vi "Index VI.vi"(6 "DBMap":refnum<class "DBMap.lvclass">, 7 "VI to analyze":path=path "C:/Projects/DMC/VISight/Source/Analyzer/Fibonacci.vi", 8 "error in (no error)":errorcluster, 9 "Valid Terminals Set":set{string}(c389)={"ControlTerminal", "OverridableParameterTerminal", "Terminal"}, 10 "AtomicSet":refnum<class "DBSet.lvclass">) -> (0 "error out":errorcluster, 3 "File Data":T1)   [LabVIEW 2020]
uses:
  DBSet/DBSet.lvclass
  DBMap/DBMap.lvclass
  <vilib>/Utility/miscctls.llb/LVMapReplaceAction.ctl
  <vilib>/Utility/traverseref.llb/VI Scripting - Traverse.lvlib
  <vilib>/Utility/traverseref.llb/TRef TravTarget.ctl
  <vilib>/security/Message Digest/API/NI_Message Digest API.lvlib
  File Metadata.ctl
  Source to Sink Array.ctl
  Node.ctl
  <vilib>/security/Message Digest/API/Instances/File/SHA-256 File Checksum.vi
  File Data.ctl
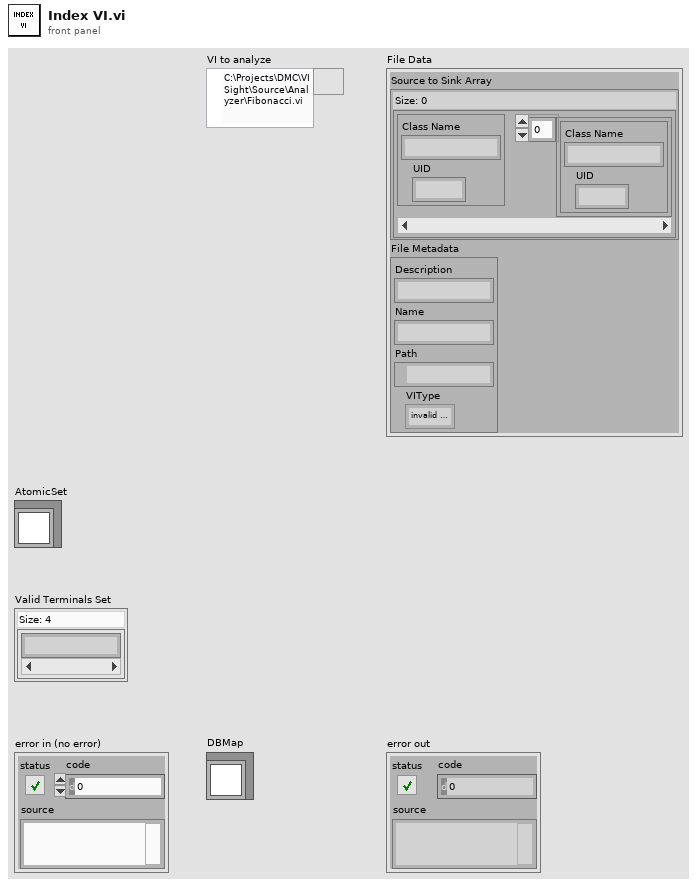
[diagram p1: front panel]
types:
  T1 = typedef "File Data.ctl" = cluster{"Source to Sink Array":T2, "File Metadata":T4}
  T2 = typedef "Source to Sink Array.ctl" = map{T3, T3[]}
  T3 = typedef "Node.ctl" = cluster{"Class Name":string, "UID":i32}
  T4 = typedef "File Metadata.ctl" = cluster{"Description":string, "Name":string, "Path":path, "VIType":enum32{"invalid VI type", "Standard VI", "Control VI", "Global VI", "Polymorphic VI", "Configuration VI", "SubSystem", "Facade VI", "Method VI", "Statechart Diagram VI"}}
  T5 = typedef "TRef TravTarget.ctl" = enum16{"FP", "BD", "Other"}
  T6 = typedef "LVMapReplaceAction.ctl" = enum32{"Modify Entry only if found", "Add or Modify Entry", "Delete Entry"}
  T7 = enum32{"invalid VI type", "Standard VI", "Control VI", "Global VI", "Polymorphic VI", "Configuration VI", "SubSystem", "Facade VI", "Method VI", "Statechart Diagram VI"}
  T8 = cluster{"ClassName":string, "Caption":string, "UID":i32}
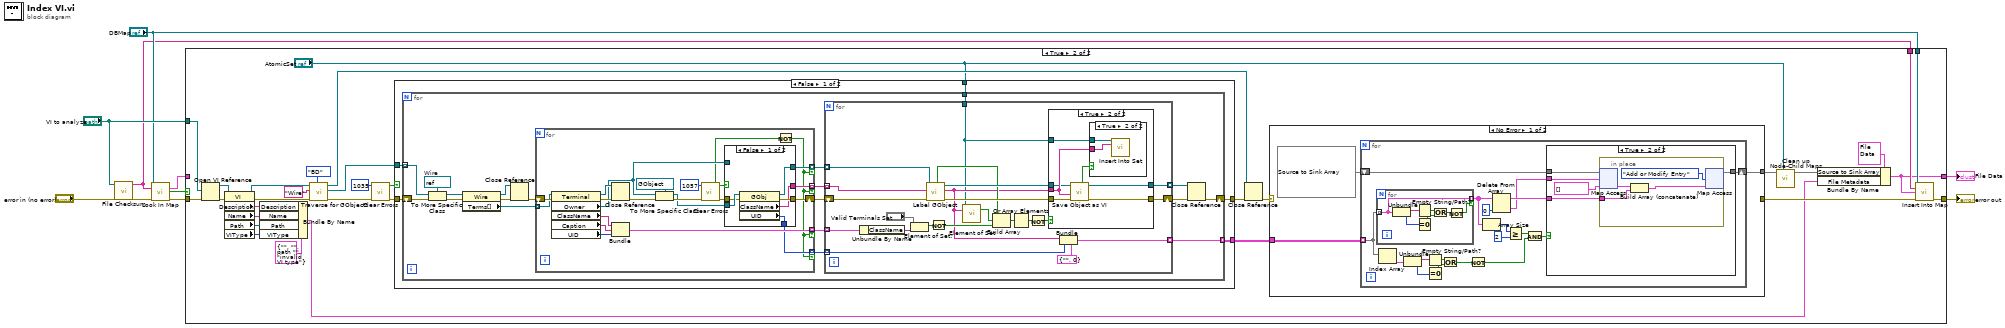
[diagram p0: block diagram]
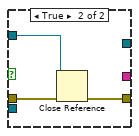
[diagram p5: hidden frame]
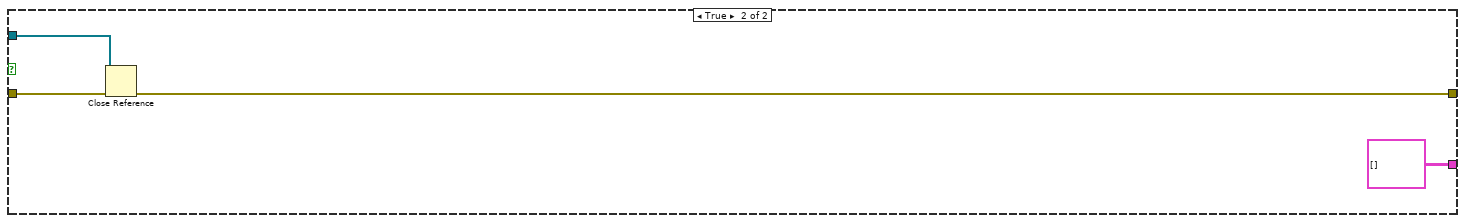
[diagram p6: hidden frame]
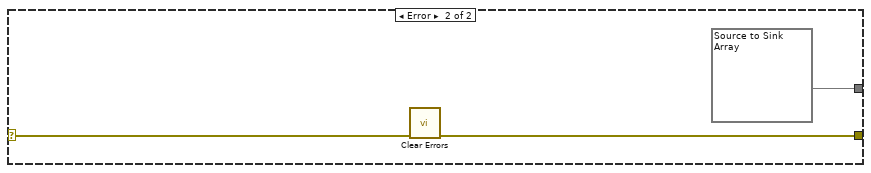
[diagram p8: hidden frame]
diagram:
  n1 = call-poly <vilib>:"File Checksum.vi"("path"="VI to analyze") -> ("digest"=w3:string)  [unwired: 9 in, 1 out]
  n2 = call "Look In Map.vi"("DBMap in"="DBMap", "Key"=w3, "error in (no error)"="error in (no error)") -> ("File Data"=w5:T1, "Not Found?"=w2:bool, "error out"=w6:errorcluster)  [unwired: 9 in, 1 out]
  n3 = case shown="True" w2 {
    tunnel: [w10 w15] -> w1
    tunnel: [w11 w34] -> w9
    tunnel: "VI to analyze" -> [_ w37]
    tunnel: w6 -> [w11 w32]
    tunnel: w5 -> [w10 _]
    tunnel: "DBMap" -> [_ w36]
    tunnel: w3 -> [_ w33]
    frame False {
    }
    frame True {
      n4 = Open VI Reference(vi path=w37, error in (no error)=w32) -> (vi reference=w21:refnum<vi>, error out=w22:errorcluster)  [unwired: 4 in]
      n5 = property class="VI"(reference=w21, error in=w22) -> (reference out=w19:refnum<vi>, error out=w20:errorcluster, "Description"=w26:string, "Name"=w25:string, "Path"=w24:path, "VIType"=w23:T7)
      n6 = Bundle By Name(cluster=T4 {"Description"="", "Name"="", "Path"=path "", "VIType"=enum."invalid VI type"} ("File Metadata"), "Description"=w26, "Name"=w25, "Path"=w24, "VIType"=w23) -> (w17:T4)
      n7 = call <vilib>:"Traverse for GObjects.vi"("Traverse Target"=TRef_TravTarget."BD", "error in (no error)"=w20, "Class Name"="Wire", "VI Refnum"=w19) -> ("error out"=w28:errorcluster, "References"=w27:refnum<vi>[], "dup VI Refnum"=w29:refnum<vi>)  [unwired: 4 in, 1 out]
      n8 = call <vilib>:"Clear Errors.vi"("error in (no error)"=w28, "specific error code to clear (0: all)"=1035) -> ("error out"=w41:errorcluster, "specific error cleared?"=w39:bool)  [unwired: 4 in]
      n9 = case shown="False" w39 {
        tunnel: [w47 w133] -> w43
        tunnel: [w46 cluster{"Class Name":string, "UID":i32}[][] []] -> w42
        tunnel: w41 -> [w45 w132]
        tunnel: w27 -> [w48 w134]
        tunnel: "AtomicSet" -> [w44 _]
        frame False {
          n10 = for {
            tunnel: w48 -> [w51] mode=indexing
            shift-right: [w55] -> w47
            shift-left: w45 -> [w54]
            tunnel: [w60] -> w46 mode=indexing
            tunnel: w44 -> [w49]
            w50 = refnum<vi> refnum  # Wire
            n11 = To More Specific Class(target class=w50, reference=w51, error in=w54) -> (specific class reference=w52:refnum<vi>, error out=w53:errorcluster)
            n12 = property on="Property Node" class="Wire"(reference=w52, error in=w53) -> (reference out=w57:refnum<vi>, error out=w59:errorcluster, "Terms[]"=w67:refnum<vi>[])
            n13 = Close Reference(reference=w57, error in (no error)=w59) -> (error out=w58:errorcluster)
            n14 = for {
              tunnel: [w103] -> w64 mode=indexing if=w101
              tunnel: [w105] -> w63 mode=indexing if=w101
              shift-right: [w104] -> w62
              shift-left: w58 -> [w121]
              tunnel: w67 -> [w119] mode=indexing
              tunnel: [w102] -> w61 mode=indexing if=w101
              tunnel: [w115] -> w65 mode=indexing if=w101
              n15 = property on="Property Node" class="Terminal"(reference=w119, error in=w121) -> (reference out=w114:refnum<vi>, error out=w113:errorcluster, "Owner"=w109:refnum<vi>, "ClassName"=w118:string, "Caption"=w117:string, "UID"=w116:i32)
              n16 = Close Reference(reference=w114, error in (no error)=w113) -> (error out=w112:errorcluster)
              n17 = Bundle("ClassName"=w118, "Caption"=w117, "UID"=w116) -> (w115:T8)  [unwired: 1 in]
              n18 = To More Specific Class(target class=refnum<vi> refnum ("reference"), reference=w109, error in=w112) -> (specific class reference=w106:refnum<vi>, error out=w111:errorcluster)
              n19 = call <vilib>:"Clear Errors.vi"("error in (no error)"=w111, "specific error code to clear (0: all)"=1057) -> ("error out"=w108:errorcluster, "specific error cleared?"=w107:bool)  [unwired: 4 in]
              n20 = case shown="False" w107 {
                tunnel: w109 -> [_ w129]
                tunnel: w108 -> [w126 w130]
                tunnel: w106 -> [w127 _]
                tunnel: [w125 _] -> w105
                tunnel: [w124 w128] -> w104
                tunnel: [w123 _] -> w103
                tunnel: [w122 _] -> w102
                frame False {
                  n21 = property class="GObj"(reference=w127, error in=w126) -> (reference out=w125:refnum<vi>, error out=w124:errorcluster, "ClassName"=w123:string, "UID"=w122:i32)
                }
                frame True {
                  n22 = Close Reference(reference=w129, error in (no error)=w130) -> (error out=w128:errorcluster)
                }
              }
              n23 = Not(x=w107) -> (.not. x?=w101:bool)
            }
            n24 = for {
              tunnel: w63 -> [w73] mode=indexing
              tunnel: w64 -> [w74] mode=indexing
              shift-right: [w85] -> w66
              shift-left: w62 -> [w76]
              tunnel: [w84] -> w56 mode=indexing
              tunnel: w65 -> [w89] mode=indexing
              tunnel: w61 -> [w87] mode=indexing
              tunnel: [w86] -> w60 mode=indexing
              tunnel: w49 -> [w68]
              n25 = Unbundle By Name(w89) -> ("ClassName"=w83:string)
              n26 = Element of Set?(10:w83, 11:"Valid Terminals Set") -> (3:w88:bool)
              n27 = call "Label GObject.vi"("error in"=w76, "GObject ClassName"=w74, "GObject Reference In"=w73) -> ("error out"=w75:errorcluster, "Label"=w70:string, "GObject Reference out"=w72:refnum<vi>, "Excluded?"=w71:bool)  [unwired: 4 in, 1 out]
              n28 = Not(x=w88) -> (.not. x?=w79:bool)
              n29 = call "Element of Set.vi"("DBSet in"=w68, "Element"=w70) -> ("Found?"=w69:bool)  [unwired: 11 in, 2 out]
              n30 = Build Array(w71, w69, w79) -> (w78:bool[])
              n31 = Or Array Elements(Boolean array=w78) -> (logical OR=w77:bool)
              n32 = Not(x=w77) -> (.not. x?=w80:bool)
              n33 = case shown="True" w80 {
                tunnel: w72 -> [w90 w94]
                tunnel: w70 -> [_ w98]
                tunnel: w75 -> [w91 w97]
                tunnel: [w91 w96] -> w85
                tunnel: [w90 w95] -> w84
                tunnel: w68 -> [_ w92]
                frame False {
                }
                frame True {
                  n34 = call "Save Object as VI.vi"("error in (no error)"=w97, "Name"=w98, "Object in"=w94) -> ("error out"=w96:errorcluster, "Object out"=w95:refnum<vi>, "Ok?"=w93:bool)  [unwired: 6 in]
                  n35 = case shown="True" w93 {
                    tunnel: w98 -> [_ w99]
                    tunnel: w92 -> [_ w100]
                    frame False {
                    }
                    frame True {
                      n36 = call "Insert Into Set.vi"("DBSet in"=w100, "Element"=w99) -> ()  [unwired: 12 in, 2 out]
                    }
                  }
                }
              }
              n37 = Bundle(cluster=cluster{"Class Name":string, "UID":i32} {"Class Name"="", "UID"=0} ("Source"), "Class Name"=w70, "UID"=w87) -> (w86:cluster{"Class Name":string, "UID":i32})
            }
            n38 = Close Reference(reference=w56, error in (no error)=w66) -> (error out=w55:errorcluster)
          }
        }
        frame True {
          n39 = Close Reference(reference=w134, error in (no error)=w132) -> (error out=w133:errorcluster)
        }
      }
      n40 = Close Reference(reference=w29, error in (no error)=w43) -> (error out=w38:errorcluster)
      n41 = case shown="No Error" w38 {
        selector: w38 -> [_ w175]
        tunnel: w42 -> [w137 _]
        tunnel: [w136 T2 {} ("Source to Sink Array")] -> w14
        tunnel: [_ w174] -> w35
        frame No Error {
          n42 = for {
            tunnel: w137 -> [w147] mode=indexing
            shift-right: [w138] -> w136
            shift-left: T2 {} ("Source to Sink Array") -> [w143]
            n43 = for {
              tunnel: w147 -> [w168] mode=indexing
              tunnel: [w168] -> w141 mode=indexing if=w166
              n44 = Unbundle(w168) -> ("Class Name"=w169:string, "UID"=w170:i32)
              n45 = Empty String/Path?(string/path=w169) -> (empty?=w171:bool)
              n46 = Equal To 0?(x=w170) -> (x = 0?=w172:bool)
              n47 = Or(x=w171, y=w172) -> (x .or. y?=w167:bool)
              n48 = Not(x=w167) -> (.not. x?=w166:bool)
            }
            n49 = Index Array(array=w147) -> (element=w150:cluster{"Class Name":string, "UID":i32})  [unwired: 1 in]
            n50 = Unbundle(w150) -> ("Class Name"=w155:string, "UID"=w154:i32)
            n51 = Empty String/Path?(string/path=w155) -> (empty?=w153:bool)
            n52 = Equal To 0?(x=w154) -> (x = 0?=w152:bool)
            n53 = Or(x=w153, y=w152) -> (x .or. y?=w151:bool)
            n54 = Not(x=w151) -> (.not. x?=w145:bool)
            n55 = Array Size(array=w141) -> (size(s)=w149:i32)
            n56 = Delete From Array(array=w141, index=0) -> (deleted portion=w139:cluster{"Class Name":string, "UID":i32}, array with subset deleted=w140:cluster{"Class Name":string, "UID":i32}[])  [unwired: 1 in]
            n57 = Greater Or Equal?(x=w149, y=2) -> (x >= y?=w146:bool)
            n58 = And(x=w146, y=w145) -> (x .and. y?=w144:bool)
            n59 = case shown="True" w144 {
              tunnel: w143 -> [w156 w160]
              tunnel: w140 -> [_ w157]
              tunnel: w139 -> [_ w158]
              tunnel: [w156 w159] -> w138
              frame False {
              }
              frame True {
                n60 = in-place {
                  in-place-border: w157 -> [w162]
                  n61 = in-place-map #1(w160, w158, cluster{"Class Name":string, "UID":i32}[] [] ("value")) -> (w165:T3[])  [unwired: 1 out]
                  n62 = Build Array (concatenate)(w165, w162) -> (w164:T3[])
                  n63 = in-place-map #1(w164, LVMapReplaceAction."Add or Modify Entry" ("action")) -> (w159:T2)  [unwired: 2 out]
                }
              }
            }
          }
        }
        frame Error {
          n64 = call <vilib>:"Clear Errors.vi"("error in (no error)"=w175) -> ("error out"=w174:errorcluster)  [unwired: 5 in, 1 out]
        }
      }
      n65 = call "Clean up Node-Child Maps.vi"("AtomicSet"="AtomicSet", "Raw Source to Sink Array"=w14) -> ("Cleaned Source to Sink Array"=w13:T2)  [unwired: 9 in]
      n66 = Bundle By Name(cluster=T1 {"Source to Sink Array"={}, "File Metadata"={"Description"="", "Name"="", "Path"=path "", "VIType"=enum."invalid VI type"}} ("File Data"), "Source to Sink Array"=w13, "File Metadata"=w17) -> (w15:T1)
      n67 = call "Insert Into Map.vi"("DBMap in"=w36, "Key"=w33, "File Data"=w15, "error in (no error)"=w35) -> ("error out"=w34:errorcluster)  [unwired: 10 in, 1 out]
    }
  }
  "error out" <- w9
  "File Data" <- w1
